vi "TestDevOnly.vi"(0 "x":dbl) -> (4 "y":dbl)   [LabVIEW 2026]
doc: "Test fixture: calls DevDep.vi."
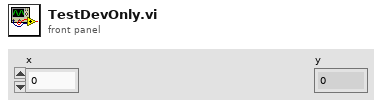
[diagram p1: front panel]
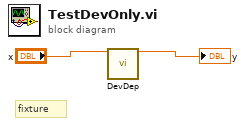
[diagram p0: block diagram]
diagram:
  # "fixture"
  n1 = call <vilib>:"DevDep.vi"("x"="x") -> ("y"=→"y":dbl)  [unwired: 14 in]
